vi "Test Rectangle Accessors.vi"(11 "error in":errorcluster) -> (15 "error out":errorcluster)   [LabVIEW 2026]
doc: "Caraya round-trip test for Rectangle\\2C generated by lvai_generate_class_test.\\0A\\0AEach case writes a value through the class's own Write accessor and reads it back through the Read accessor\\2C both called as ORDINARY STATIC SUBVIS. AIXML cannot author a class-typed terminal\\2C so the calls were generated against sockets and swapped for the real accessors with LabVIEW's own Replace\\2C which re-types the wires.\\0A\\0AThe error cluster carries the FIRST failure only. Read the JUnit report for all of them."
uses:
  <vilib>/addons/_JKI Toolkits/Caraya/classes/Test/Test.lvclass
  <vilib>/addons/_JKI Toolkits/Caraya/classes/Assert/Assert.lvclass
  Rectangle/Rectangle.lvclass
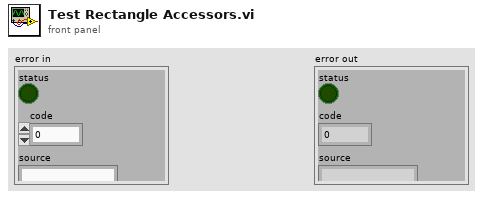
[diagram p1: front panel]
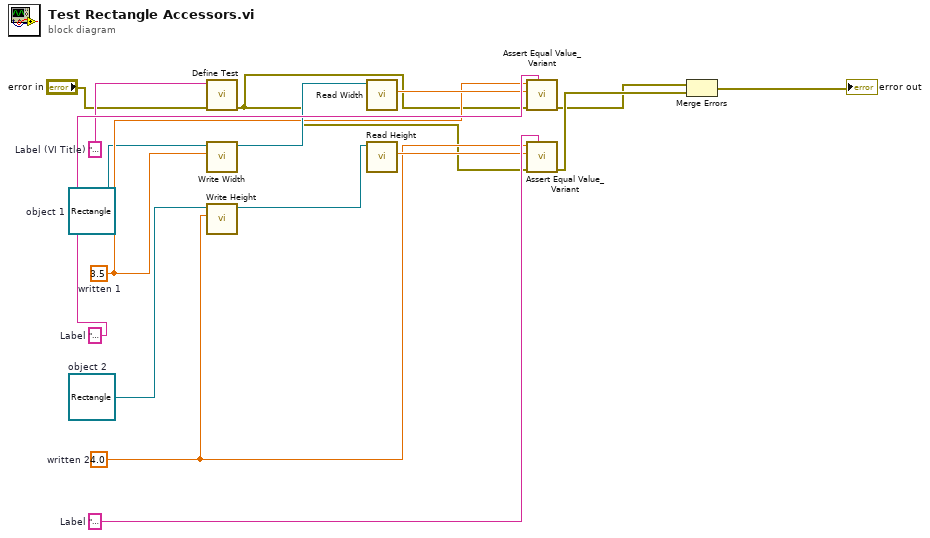
[diagram p0: block diagram]
diagram:
  w14 = "Height round trip"  # Label
  w11 = 4.0  # written 2
  w10 = refnum<class "Rectangle.lvclass"> refnum  # object 2
  w8 = "Width round trip"  # Label
  w5 = 3.5  # written 1
  w4 = refnum<class "Rectangle.lvclass"> refnum  # object 1
  w2 = "Test Rectangle Accessors"  # Label (VI Title)
  n1 = call <vilib>:"Define Test.vi"("error in (no error)"="error in", "Label (VI Title)"=w2) -> ("error out"=w3:errorcluster)  [unwired: 8 in, 1 out]
  n2 = call-dynamic "Write Width.vi"("Width"=w5, "Rectangle in"=w4) -> ("Rectangle out"=w6:refnum<class "Rectangle.lvclass">)  [unwired: 8 in, 1 out]
  n3 = call-dynamic "Write Height.vi"("Height"=w11, "Rectangle in"=w10) -> ("Rectangle out"=w12:refnum<class "Rectangle.lvclass">)  [unwired: 8 in, 1 out]
  n4 = call-dynamic "Read Width.vi"("Rectangle in"=w6) -> ("Width"=w7:dbl)  [unwired: 8 in, 2 out]
  n5 = call-dynamic "Read Height.vi"("Rectangle in"=w12) -> ("Height"=w13:dbl)  [unwired: 8 in, 2 out]
  n6 = call <vilib>:"Assert Equal Value_Variant.vi"("Label"=w8, "error in (no error)"=w3, "Actual"=w7, "Expected"=w5) -> ("error out"=w9:errorcluster)  [unwired: 6 in, 1 out]
  n7 = call <vilib>:"Assert Equal Value_Variant.vi"("Label"=w14, "error in (no error)"=w3, "Actual"=w13, "Expected"=w11) -> ("error out"=w15:errorcluster)  [unwired: 6 in, 1 out]
  n8 = Merge Errors(w9, w15) -> (→"error out":errorcluster)
